vi "PicoScopeospaGetValues.vi"(7 "Buffer and Transfer Settings":T1={"startIndex"=0, "Samples"=1000, "Down Sample Ratio"=1, "Down-Sample Mode"=1} {"Down-Sample Mode" items=["RAW none"=2147483648, "None"=0, "Aggregate"=1, "Decimate"=2, "Average"=4]; "Down Sample Ratio" step=1; "Samples" format="%_6p"}, 8 "error in (no error)":errorcluster, 11 "handle in":i16) -> (0 "error out":errorcluster, 3 "handle out":i16, 4 "overflow":i16 format="%010b", 6 "noOfSamples":u64)   [LabVIEW 2010]
doc: "Calls GetValues"
uses:
  psospa.dll
  shared/Buffer and Transfer Settings.ctl
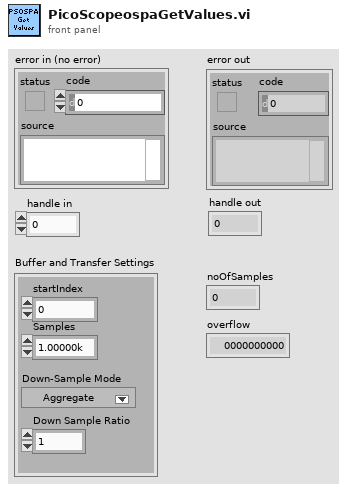
[diagram p1: front panel]
types:
  T1 = typedef "Buffer and Transfer Settings.ctl" = cluster{"startIndex":u64, "Samples":u64, "Down Sample Ratio":u64, "Down-Sample Mode":u32}
  T2 = cluster{"status":bool, "code":u32, "source":string}
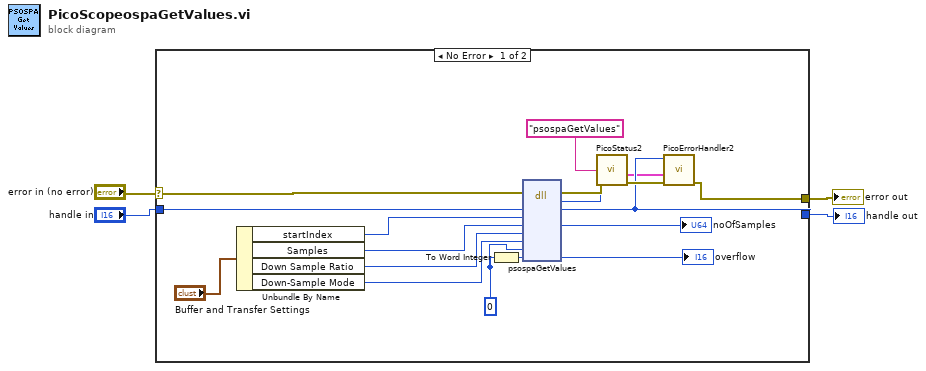
[diagram p0: block diagram]
diagram:
  n1 = case shown="No Error" "error in (no error)" {
    selector: "error in (no error)" -> [w10 w23]
    tunnel: "handle in" -> [w9 w24]
    tunnel: [w7 w24] -> w4
    tunnel: [w8 w23] -> w3
    frame No Error {
      w14 = u64 0 ("overflow")
      n2 = Unbundle By Name("Buffer and Transfer Settings") -> ("startIndex"=w11:u64, "Samples"=w22:u64, "Down Sample Ratio"=w18:u64, "Down-Sample Mode"=w19:u32)
      n3 = To Word Integer(number=w14) -> (16bit integer=w20:i16)
      n4 = dll-call lib="psospa.dll" fn="psospaGetValues" ("ps3000.dll:_ps3000_open_unit@0")(error in=w10, "handle"=w9, "startIndex"=w11, "noOfSamples"=w22, "downSampleRatio"=w18, "downSampleRatioMode"=w19, "segmentIndex"=w14, "overflow"=w20) -> (error out=w17:errorcluster, "PICO_STATUS"=w16:u32, "handle"=w7:i16, "noOfSamples"=→"noOfSamples":u64, "overflow"=→"overflow":i16)  [unwired: 6 in, 1 out]
      n5 = call "PicoStatus2.vi"("PICO source"="psospaGetValues" ("source"), "Error in"=w17, "PICO STATUS"=w16) -> ("error out"=w21:errorcluster, "PICO_STATUS out"=w5:T2)  [unwired: 5 in]
      n6 = call "PicoErrorHandler2.vi"("error in (no error)"=w21, "PICO_STATUS in"=w5, "handle In"=w7) -> ("error out"=w8:errorcluster)  [unwired: 8 in]
    }
    frame Error {
    }
  }
  "error out" <- w3
  "handle out" <- w4
